vi "Create Map from Translations.vi"(1 "Translations":T1[](array[typedef])) -> (0 "Map out":map{string, T4}(c390))   [LabVIEW 2019, in "Language Editor.lvlib"]
doc: "- - -\nCopyright (c) 2026, Merecs Engineering GmbH"
uses:
  Language Editor.lvlib
  type defs/Cluster Translations.ctl
  Language Selection/TypeDefs/Cluster PropertyTranslation.ctl
  Language Selection/TypeDefs/Enum Property Type.ctl
  Language Selection/TypeDefs/Cluster Language.ctl
  Language Selection/Language Selection.lvlib
panel:
  # "Connector Pane"
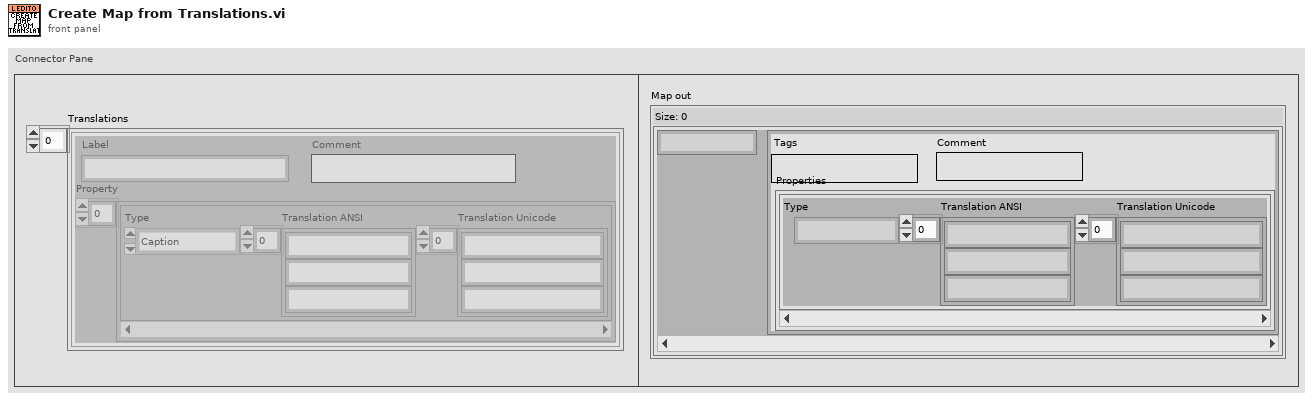
[diagram p1: front panel]
types:
  T1 = typedef "Language Selection.lvlib/Cluster Language.ctl" = cluster{"Label":string, "Comment":string, "Property":T2[]}
  T2 = typedef "Language Selection.lvlib/Cluster PropertyTranslation.ctl" = cluster{"Type":T3, "Translation ANSI":string[], "Translation Unicode":string[]}
  T3 = typedef "Language Selection.lvlib/Enum Property Type.ctl" = enum16{"NA", "Caption", "String Value", "Boolean Text", "Ring Strings", "1D Array Elements", "2D Array Elements", "(MC)Listbox Header", "(MC)Listbox Items", "Tab Pages Names", "X & Y GraphChart", "Plot Names", "Table Headers", "Table Items", "TipStrip", "Combobox Strings", "Cursor Name", "Tree Col Headers"}
  T4 = typedef "Language Editor.lvlib/Cluster Translations.ctl" = cluster{"Tags":string, "Comment":string, "Properties":T2[]}
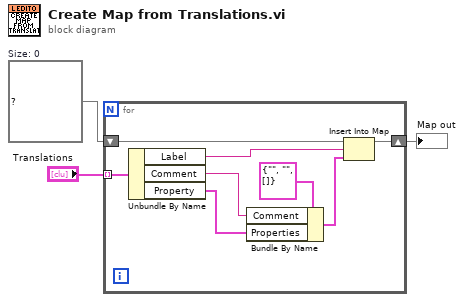
[diagram p0: block diagram]
diagram:
  w1 = map{string, T4} {}  # Size: 0
  n1 = for {
    shift-right: [w10] -> w3
    shift-left: w1 -> [w11]
    tunnel: "Translations" -> [w9] mode=indexing
    n2 = Unbundle By Name(w9) -> ("Label"=w8:string, "Comment"=w6:string, "Property"=w5:T2[])
    n3 = Bundle By Name(cluster=T4 {"Tags"="", "Comment"="", "Properties"=[]} ("Translation"), "Comment"=w6, "Properties"=w5) -> (w4:T4)
    n4 = Insert Into Map(map in=w11, key=w8, value=w4) -> (map out=w10:map{string, T4})  [unwired: 2 out]
  }
  "Map out" <- w3
